vi "DSS-test-bilinear.vi"(8 "error in":errorcluster) -> (0 "error out":errorcluster)   [LabVIEW 2020, in "DSS-Tests.lvlib"]
doc: "Caraya test of RDC-permittivity-Bilinear on aff_22p5c_ethanol-48 with the simulated open, DI water and salt water standards at 22.5 C: Common Format out against its golden file, and Permativity' and Permativity'' against the independent Python reference."
uses:
  DSS-Tests.lvlib
  <vilib>/addons/_JKI Toolkits/Caraya/classes/Test/Test.lvclass
  Reflector/RFH-Reflection_File_Handler.lvlib
  Computation/RDC-Reflection_Data_Computation.lvlib
  <vilib>/addons/_JKI Toolkits/Caraya/classes/Assert/Assert.lvclass
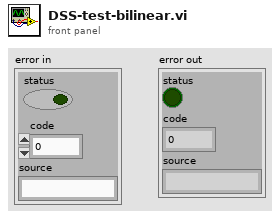
[diagram p1: front panel]
types:
  T1 = typedef "RFH-Reflection_File_Handler.lvlib/RFH-common_data_format.ctl" = cluster{"Frequency":dbl[], "Reflection'":dbl[], "Reflection''":dbl[], "Permativity'":dbl[], "Permativity''":dbl[], "Conductivity":dbl[], "Loss Tangent":dbl[], "Resistance":dbl[], "Reactance":dbl[]}
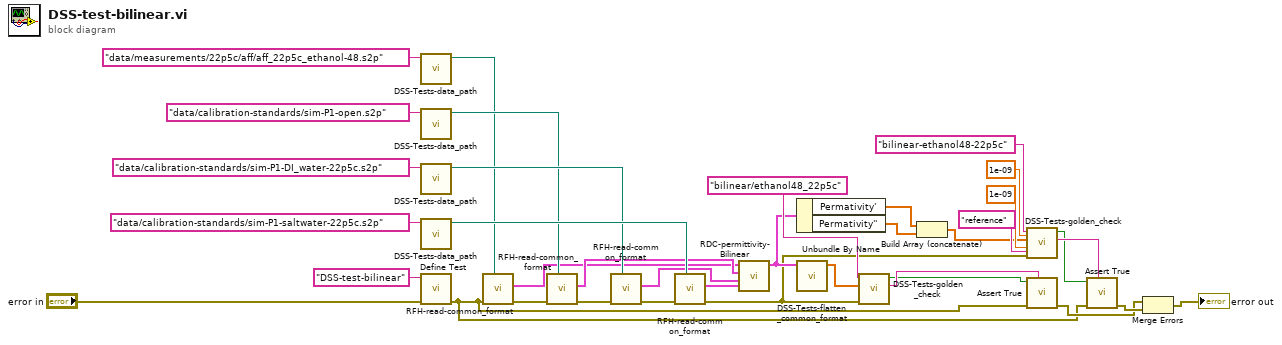
[diagram p0: block diagram]
diagram:
  n1 = call "DSS-Tests-data_path.vi"("relative path"="data/measurements/22p5c/aff/aff_22p5c_ethanol-48.s2p") -> ("path"=w5:path)  [unwired: 10 in]
  n2 = call "DSS-Tests-data_path.vi"("relative path"="data/calibration-standards/sim-P1-open.s2p") -> ("path"=w9:path)  [unwired: 10 in]
  n3 = call "DSS-Tests-data_path.vi"("relative path"="data/calibration-standards/sim-P1-DI_water-22p5c.s2p") -> ("path"=w13:path)  [unwired: 10 in]
  n4 = call "DSS-Tests-data_path.vi"("relative path"="data/calibration-standards/sim-P1-saltwater-22p5c.s2p") -> ("path"=w17:path)  [unwired: 10 in]
  n5 = call <vilib>:"Define Test.vi"("error in (no error)"="error in", "Label (VI Title)"="DSS-test-bilinear") -> ("error out"=w3:errorcluster)  [unwired: 8 in, 1 out]
  n6 = call "RFH-read-common_format.vi"("file path (dialog if empty)"=w5, "error in"=w3) -> ("error out"=w6:errorcluster, "Common Format"=w7:T1)  [unwired: 8 in]
  n7 = call "RFH-read-common_format.vi"("file path (dialog if empty)"=w9, "error in"=w6) -> ("error out"=w10:errorcluster, "Common Format"=w11:T1)  [unwired: 8 in]
  n8 = call "RFH-read-common_format.vi"("file path (dialog if empty)"=w13, "error in"=w10) -> ("error out"=w14:errorcluster, "Common Format"=w15:T1)  [unwired: 8 in]
  n9 = call "RFH-read-common_format.vi"("file path (dialog if empty)"=w17, "error in"=w14) -> ("error out"=w18:errorcluster, "Common Format"=w19:T1)  [unwired: 8 in]
  n10 = call "RDC-permittivity-Bilinear.vi"("Salt Water"=w19, "DI-Water"=w15, "Open/Air"=w11, "Common Format"=w7) -> ("Common Format out"=w20:T1)  [unwired: 7 in]
  n11 = Unbundle By Name(w20) -> ("Permativity'"=w26:dbl[], "Permativity''"=w27:dbl[])
  n12 = call "DSS-Tests-flatten_common_format.vi"("Common Format"=w20) -> ("flat"=w21:dbl[])  [unwired: 10 in]
  n13 = call "DSS-Tests-golden_check.vi"("error in"=w18, "actual"=w21, "golden name"="bilinear/ethanol48_22p5c") -> ("message"=w24:string, "pass"=w23:bool)  [unwired: 6 in, 1 out]
  n14 = Build Array (concatenate)(w26, w27) -> (w28:dbl[])
  n15 = call "DSS-Tests-golden_check.vi"("folder"="reference", "abs tol"=1e-09, "error in"=w18, "rel tol"=1e-09, "actual"=w28, "golden name"="bilinear-ethanol48-22p5c") -> ("message"=w34:string, "pass"=w33:bool)  [unwired: 3 in, 1 out]
  n16 = call <vilib>:"Assert True.vi"("Label"=w24, "error in (no error)"=w3, "True?"=w23) -> ("error out"=w25:errorcluster)  [unwired: 7 in, 1 out]
  n17 = call <vilib>:"Assert True.vi"("Label"=w34, "error in (no error)"=w3, "True?"=w33) -> ("error out"=w35:errorcluster)  [unwired: 7 in, 1 out]
  n18 = Merge Errors(w25, w35) -> (→"error out":errorcluster)
